vi "ResetDevice.vi"(8 "error in":errorcluster) -> (0 "error out":errorcluster)   [LabVIEW 2020, in "OpenLvVision_OpenCv.lvlib" / "Cuda.lvlib"]
doc: "Explicitly destroys and cleans up all resources associated with the current device in the current process."
uses:
  Cuda.lvlib
  OpenLvVision_OpenCv.lvlib
  <vilib>/Utility/error.llb/Error Cluster From Error Code.vi
  <vilib>/ErrorRing/Error Ring.xnode
  Dlls/OlvOpenCvWrapper.dll
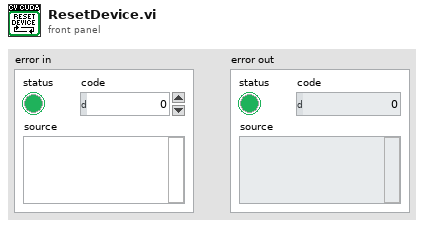
[diagram p1: front panel]
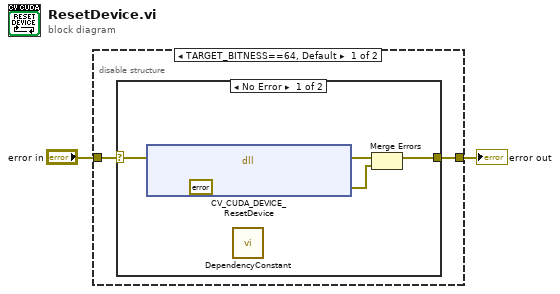
[diagram p0: block diagram]
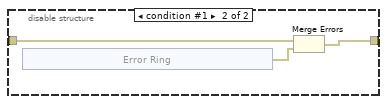
[diagram p3: hidden frame]
diagram:
  n1 = disable-structure shown="TARGET_BITNESS==64, Default" {
    disable-tunnel: "error in" -> [w3 w13]
    disable-tunnel: [w4 w12] -> w1
    frame condition #0 (active) {
      n2 = case shown="No Error" w3 {
        selector: w3 -> [w5 w10]
        tunnel: [w6 w10] -> w4
        frame No Error {
          n3 = dll-call lib="C:/Users/lukas/Documents/OpenLvVision_OpenCv/SourceCode/LabView/OpenLvVision_OpenCv/Dlls/OlvOpenCvWrapper.dll" fn="CV_CUDA_DEVICE_ResetDevice"(error in=w5, "Error"=errorcluster {"status"=FALSE, "code"=0, "source"=""} ("error out")) -> (error out=w9:errorcluster, "Error"=w8:errorcluster)  [unwired: 3 in, 1 out]
          n4 = call "DependencyConstant.vi"() -> ()  [unwired: 12 in]
          n5 = Merge Errors(w9, w8) -> (w6:errorcluster)
        }
        frame Error {
        }
      }
    }
    frame condition #1 {
      n6 = xnode "Error Ring"() -> ("error out"=w11:errorcluster)
      n7 = Merge Errors(w13, w11) -> (w12:errorcluster)
    }
  }
  "error out" <- w1
